vi "Check Prompt Arguments.vi"(8 "error in":errorcluster, 9 "id":i32, 10 "message json":string, 11 "arguments json":string) -> (0 "error out":errorcluster, 3 "arguments json out":string)   [LabVIEW 2020, in "MCP Server.lvlib"]
doc: "Prepares the arguments of prompts/get.\n\narguments is optional in MCP: if the request has none, arguments json out is an empty object, so a prompt without required arguments works.\nIf the prompt has required arguments that the request does not give, error out is LabVIEW error 402841 (the code JSONtext uses for a missing item) with the names of the missing arguments. Build Error Response.vi turns that into JSON-RPC error -32602."
uses:
  MCP Server.lvlib
  c38156dc-efef-49bc-98a5-8be9433653da.vi
  30c229a7-cefd-464f-a6be-24ed288cced7.vi
  a6e75a6f-32b0-48fe-86cd-c0e493bcd1f6.vi
  <vilib>/JDP Science/JSONtext/Next JSON Value.vi
  <vilib>/JDP Science/JSONtext/String Subset.vi
  <vilib>/JDP Science/JSONtext/Parsing/Advance past next JSON Value (inlined COPY).vi
  <vilib>/JDP Science/JSONtext/Parsing/Advance past whitespace.vi
  <vilib>/JDP Science/JSONtext/Parsing/Advance past String.vi
  <vilib>/JDP Science/JSONtext/Parsing/Advance past Number.vi
  <vilib>/JDP Science/JSONtext/Parsing/Advance past Line Ending.vi
  <vilib>/JDP Science/JSONtext/Parsing/Parse Full Path or Item Name.vi
  <vilib>/JDP Science/JSONtext/Parsing/Advance past Array.vi
  <vilib>/JDP Science/JSONtext/Parsing/Advance past Object.vi
  <vilib>/JDP Science/JSONtext/support/Error Cluster From Code.vi
  <vilib>/JDP Science/JSONtext/Offset/Find Item Locations by Path.vi
  <vilib>/JDP Science/JSONtext/JSON text to Variant.vi
  <vilib>/JDP Science/JSONtext/Variant to JSON Text.vi
  <vilib>/JDP Science/JSONtext/LVClass Serializer/JSONtext LVClass Serializer.lvclass
  <vilib>/JDP Science/JSONtext/JSONtext.lvlib
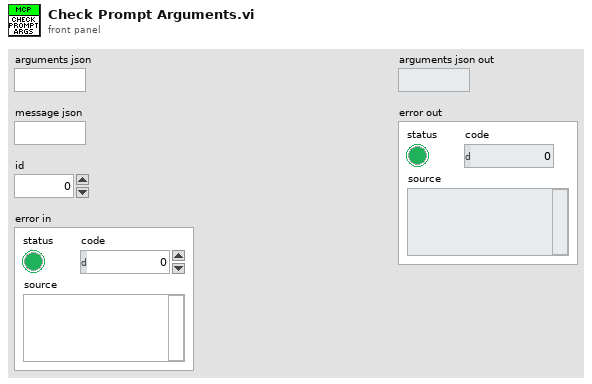
[diagram p1: front panel]
types:
  T1 = typedef "MCP Server.lvlib/Prompt Data.ctl" = cluster{"name":string, "description":string, "arguments":T2[], "return terminal name":string, "results description":string, "VI Refnum":refnum<vi>}
  T2 = typedef "MCP Server.lvlib/Prompt Argument.ctl" = cluster{"name":string, "description":string, "required":bool, "raw_name":string}
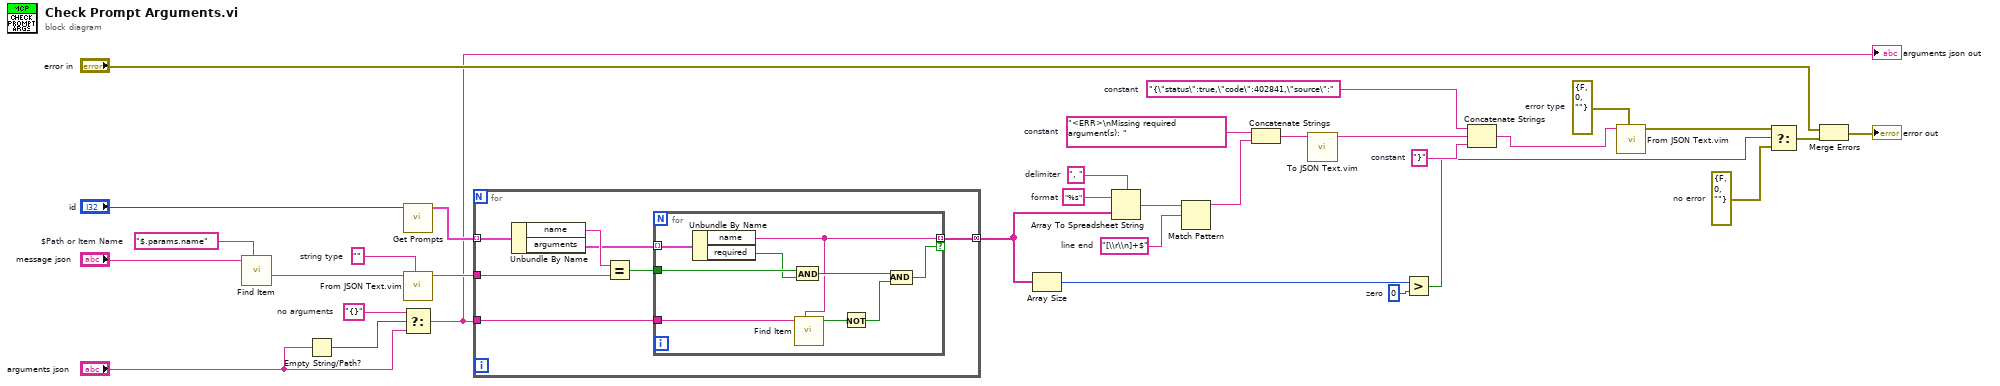
[diagram p0: block diagram]
diagram:
  w5 = errorcluster {"status"=FALSE, "code"=0, "source"=""}  # no error
  w8 = errorcluster {"status"=FALSE, "code"=0, "source"=""}  # error type
  w10 = "}"  # constant
  w12 = "{\"status\":true,\"code\":402841,\"source\":"  # constant
  w15 = "<ERR>\nMissing required argument(s): "  # constant
  w16 = "[\\r\\n]+$"  # line end
  w18 = ", "  # delimiter
  w20 = "%s"  # format
  w21 = 0  # zero
  w26 = ""  # string type
  w28 = "$.params.name"  # $Path or Item Name
  w32 = "{}"  # no arguments
  n1 = call <vilib>:"Find Item.vi"("$Path or Item Name"=w28, "JSON"="message json") -> ("<JSON>"=w27:string)  [unwired: 6 in, 3 out]
  n2 = Empty String/Path?(string/path="arguments json") -> (empty?=w31:bool)
  n3 = call "Get Prompts.vi"("id"="id") -> ("Prompts"=w24:T1[])  [unwired: 9 in, 1 out]
  n4 = call "From JSON Text.vim"("Data Type and Default Value"=w26, "JSON"=w27) -> ("Data out"=w23:string)  [unwired: 8 in, 1 out]
  n5 = Select(t=w32, s=w31, f="arguments json") -> (s? t:f=w2:string)
  "arguments json out" <- w2
  n6 = for {
    tunnel: w24 -> [w39] mode=indexing
    tunnel: w23 -> [w37]
    tunnel: w2 -> [w34]
    tunnel: [w33] -> w19 mode=concatenating
    n7 = Unbundle By Name(w39) -> ("name"=w38:string, "arguments"=w36:T2[])
    n8 = Equal?(x=w38, y=w37) -> (x = y?=w35:bool)
    n9 = for {
      tunnel: w36 -> [w48] mode=indexing
      tunnel: w35 -> [w45]
      tunnel: w34 -> [w47]
      tunnel: [w40] -> w33 mode=indexing if=w41
      n10 = Unbundle By Name(w48) -> ("name"=w40:string, "required"=w44:bool)
      n11 = And(x=w45, y=w44) -> (x .and. y?=w43:bool)
      n12 = call <vilib>:"Find Item.vi"("$Path or Item Name"=w40, "JSON"=w47) -> ("Found"=w46:bool)  [unwired: 6 in, 3 out]
      n13 = Not(x=w46) -> (.not. x?=w42:bool)
      n14 = And(x=w43, y=w42) -> (x .and. y?=w41:bool)
    }
  }
  n15 = Array Size(array=w19) -> (size(s)=w22:i32)
  n16 = Array To Spreadsheet String(delimiter (Tab)=w18, array=w19, 3:w20) -> (spreadsheet string=w17:string)
  n17 = Match Pattern(string=w17, regular expression=w16) -> (before substring=w14:string)  [unwired: 1 in, 3 out]
  n18 = Concatenate Strings(w15, w14) -> (w13:string)
  n19 = call "To JSON Text.vim"("Anything"=w13) -> ("<JSON>"=w11:string)  [unwired: 9 in, 1 out]
  n20 = Greater?(x=w22, y=w21) -> (0:w6:bool)
  n21 = Concatenate Strings(w12, w11, w10) -> (w9:string)
  n22 = call "From JSON Text.vim"("Data Type and Default Value"=w8, "JSON"=w9) -> ("Data out"=w7:errorcluster)  [unwired: 8 in, 1 out]
  n23 = Select(t=w7, s=w6, f=w5) -> (s? t:f=w3:errorcluster)
  n24 = Merge Errors("error in", w3) -> (→"error out":errorcluster)
